vi "Query.vi"(5 "buffered":bool=TRUE, 6 "commandTimeout":i32=-1, 7 "CommandType":i32(ring)=-1 items=["Text"=1, "StoredProcedure"=4, "TableDirect"=512], 8 "error in (no error)":errorcluster, 9 "DynamicParameters":refnum<class "DynamicParameters.lvclass">, 10 "sql":string, 11 "PGJDPMapper in":refnum<class "Mapper.lvclass">) -> (0 "error out":errorcluster, 2 "Query Result out":refnum<class "Query Result.lvclass">, 3 "PGJDPMapper out":refnum<class "Mapper.lvclass">)   [LabVIEW 2020, in "ORM_pgsql_jdp.lvlib" / "Mapper.lvclass"]
uses:
  Mapper.lvclass
  C:/Program Files/National Instruments/LabVIEW 2020/vi.lib/Viviota/shared/ORM.lvlibp/SqlMapper/SqlMapper.lvclass
  <vilib>/Viviota/shared/ORM.lvlibp/Query Result/Query Result.lvclass
  <vilib>/Viviota/shared/ORM.lvlibp/DynamicParameters/DynamicParameters.lvclass
  dbc/DBC.lvclass
  PGJDPParameter/Parameter.lvclass
  C:/Program Files/National Instruments/LabVIEW 2020/vi.lib/Viviota/shared/ORM.lvlibp/DynamicParameters/DynamicParameters.lvclass
  PGJDPResult/Result.lvclass
  C:/Program Files/National Instruments/LabVIEW 2020/vi.lib/Viviota/shared/ORM.lvlibp/Query Result/Query Result.lvclass
  <vilib>/Viviota/shared/ORM.lvlibp/SqlMapper/Read DbConnection.vi
  dbc/Read Connection.vi
  <vilib>/Viviota/shared/ORM.lvlibp/DynamicParameters/Read ParameterNames.vi
  <vilib>/Viviota/shared/ORM.lvlibp/DynamicParameters/Read ParameterValues.vi
  <vilib>/JDP Science/PostgreSQL Library/Connection/Execute Command (Result).vi
  <vilib>/Viviota/shared/ORM.lvlibp/DbConnection/DbConnection.lvclass
  <vilib>/JDP Science/PostgreSQL Library/Connection/PQ Connection.lvclass
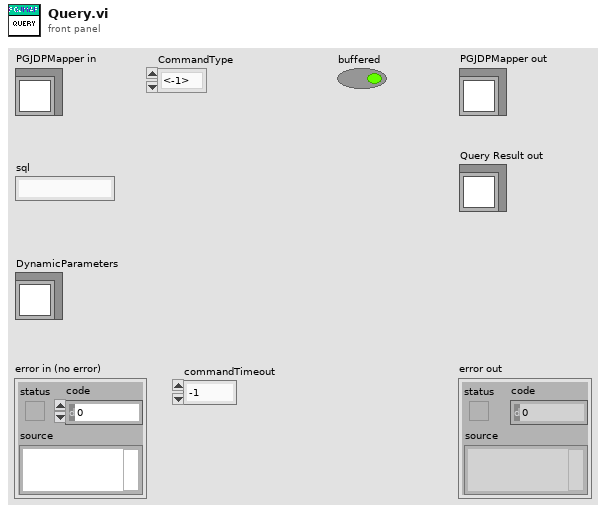
[diagram p1: front panel]
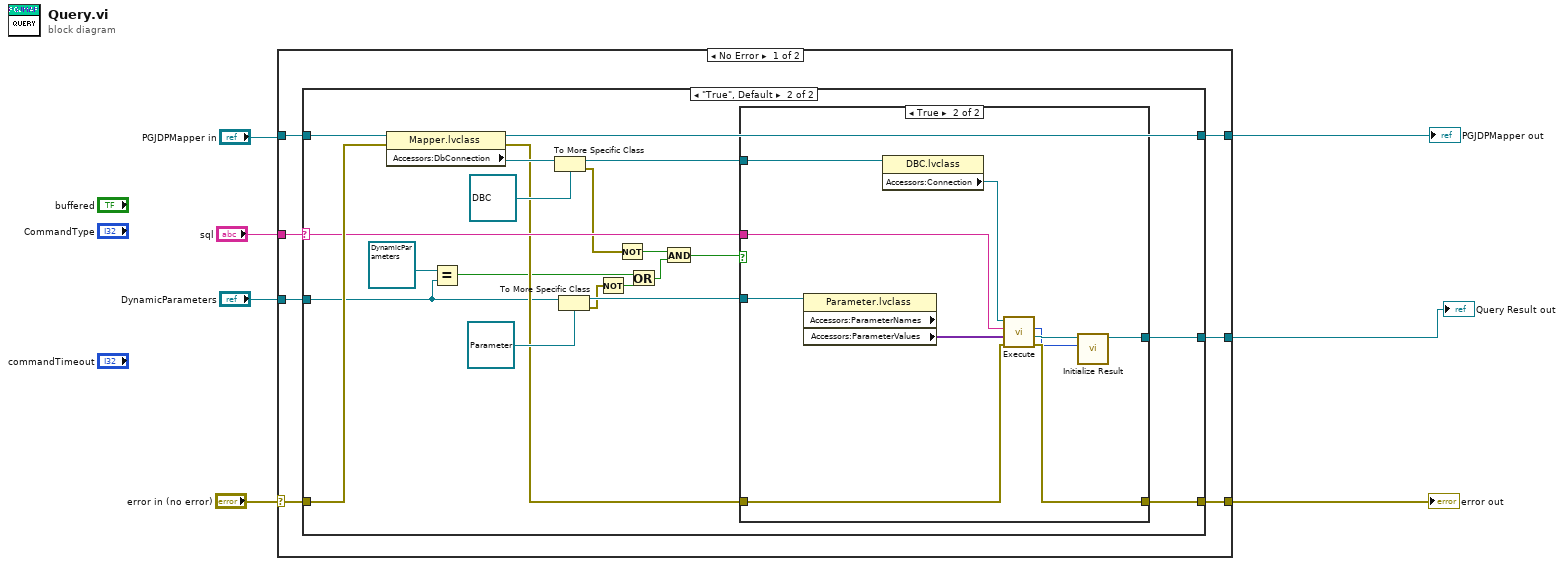
[diagram p0: block diagram]
diagram:
  n1 = case shown="No Error" "error in (no error)" {
    selector: "error in (no error)" -> [w12 w50]
    tunnel: "PGJDPMapper in" -> [w14 w49]
    tunnel: [w13 w49] -> w6
    tunnel: [w11 w50] -> w2
    tunnel: "sql" -> [w10 _]
    tunnel: "DynamicParameters" -> [w9 _]
    tunnel: [w8 _] -> w1
    frame No Error {
      n2 = case shown="\"True\", Default" w10 {
        selector: w10 -> [_ w30]
        tunnel: w14 -> [w16 w37]
        tunnel: [w16 w36] -> w13
        tunnel: w12 -> [w15 w35]
        tunnel: [w15 w27] -> w11
        tunnel: w9 -> [_ w18]
        tunnel: [_ w26] -> w8
        frame "" {
        }
        frame "True", Default {
          n3 = property class="Mapper.lvclass"(reference=w37, error in=w35) -> (reference out=w36:refnum<class "Mapper.lvclass">, error out=w28:errorcluster, "Accessors:DbConnection"=w34:refnum<class "DbConnection.lvclass">)
          n4 = Equal?(x=refnum<class "DynamicParameters.lvclass"> refnum ("DynamicParameters"), y=w18) -> (x = y?=w23:bool)
          n5 = To More Specific Class(target class=refnum<class "DBC.lvclass"> refnum ("ORM_pgsql_jdp.lvlib:DBC.lvclass"), reference=w34) -> (specific class reference=w29:refnum<class "DBC.lvclass">, error out=w20:errorcluster)  [unwired: 1 in]
          n6 = To More Specific Class(target class=refnum<class "Parameter.lvclass"> refnum ("ORM_pgsql_jdp.lvlib:PGJDPParameter.lvclass"), reference=w18) -> (specific class reference=w31:refnum<class "Parameter.lvclass">, error out=w19:errorcluster)  [unwired: 1 in]
          n7 = Not(x=w19) -> (.not. x?=w24:bool)
          n8 = Not(x=w20) -> (.not. x?=w21:bool)
          n9 = Or(x=w23, y=w24) -> (x .or. y?=w22:bool)
          n10 = And(x=w21, y=w22) -> (x .and. y?=w17:bool)
          n11 = case shown="True" w17 {
            tunnel: w31 -> [_ w48]
            tunnel: w30 -> [_ w46]
            tunnel: w29 -> [_ w45]
            tunnel: w28 -> [w38 w43]
            tunnel: [w38 w42] -> w27
            tunnel: [_ w39] -> w26
            frame False {
            }
            frame True {
              n12 = property class="Parameter.lvclass" props=["Accessors:ParameterNames", "Accessors:ParameterValues"](reference=w48) -> ("Accessors:ParameterValues"=w47:variant[])  [unwired: 1 in, 3 out]
              n13 = property class="DBC.lvclass"(reference=w45) -> ("Accessors:Connection"=w44:refnum<class "PQ Connection.lvclass">)  [unwired: 1 in, 2 out]
              n14 = call-poly <vilib>:"Execute.vi"("error in (no error)"=w43, "Parameter(s)"=w47, "SQL"=w46, "PQ Connection in"=w44) -> ("error out"=w42:errorcluster, "PQ Result"=w41:refnum<class "PQ Result.lvclass">, "Number of Rows"=w40:i32)  [unwired: 4 in, 1 out]
              n15 = call "Initialize Result.vi"("Count"=w40, "PQ Result"=w41) -> ("PGJDPResult out"=w39:refnum<class "Result.lvclass">)  [unwired: 8 in, 1 out]
            }
          }
        }
      }
    }
    frame Error {
    }
  }
  "error out" <- w2
  "PGJDPMapper out" <- w6
  "Query Result out" <- w1
